vi "Engine-UpdateLayout.vi"(8 "error in (no error)":errorcluster, 11 "GLF Window in":refnum<class "Window.lvclass">) -> (0 "error out":errorcluster, 3 "GLF Window out":refnum<class "Window.lvclass">)   [LabVIEW 2020, in "GLF.lvlib" / "Window.lvclass"]
uses:
  Window.lvclass
  Window.lvclass/Window.ctl
  IAmVIEW/IAmVIEW.lvclass
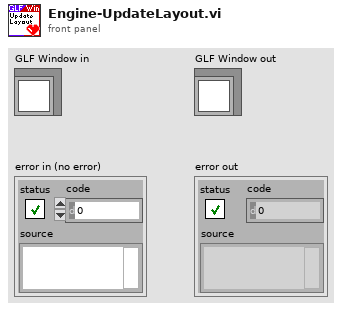
[diagram p1: front panel]
types:
  T1 = typedef "GLF.lvlib/Window.lvclass/DVR--cluster.ctl" = cluster{"SDL_Window *":T2, "Window ID":T3, "SDL_Renderer *":T4, "Event Interface":refnum<class "WindowEventInterface.lvclass">, "VIEW":refnum<class "IAmVIEW.lvclass">, "Flags":T5}
  T2 = typedef "SDL3.lvlib/Video.lvlib/SDL_Window--pointer.ctl" = i64
  T3 = typedef "SDL3.lvlib/Video.lvlib/WindowID--integer.ctl" = u32
  T4 = typedef "SDL3.lvlib/Render.lvlib/SDL_Renderer--pointer.ctl" = i64
  T5 = typedef "GLF.lvlib/Window.lvclass/Flags--cluster.ctl" = cluster{"VIEW Needs Render":bool}
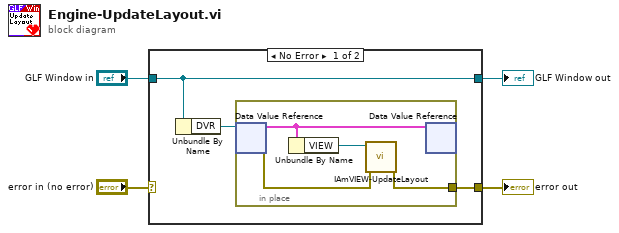
[diagram p0: block diagram]
diagram:
  n1 = case shown="No Error" "error in (no error)" {
    selector: "error in (no error)" -> [_ w13]
    tunnel: [w5 w13] -> w3
    tunnel: [w7 w12] -> w1
    tunnel: "GLF Window in" -> [w7 w12]
    frame No Error {
      n2 = Unbundle By Name(w7) -> ("DVR"=w6:refnum<data-value>)
      n3 = in-place {
        in-place-border: [w8] -> w5
        n4 = in-place-dvr #1(w6) -> (w10:T1, w9:errorcluster)
        n5 = Unbundle By Name(w10) -> ("VIEW"=w11:refnum<class "IAmVIEW.lvclass">)
        n6 = call-dynamic "IAmVIEW-UpdateLayout.vi"("error in (no error)"=w9, "IAmVIEW in"=w11) -> ("error out"=w8:errorcluster)  [unwired: 8 in, 1 out]
        n7 = in-place-dvr #1(w10) -> ()  [unwired: 2 out]
      }
    }
    frame Error {
    }
  }
  "error out" <- w3
  "GLF Window out" <- w1
